vi "subvi(name).vi"(8 "error in":errorcluster) -> (0 "error out":errorcluster, 2 "Button 2":bool, 3 "Cluster ind":T1)   [LabVIEW 2025]
uses:
  Cluster(ctrl2).ctl
  c1a9ddd9-b479-4c69-873f-00e1aee4619d.vi
panel:
  in  "Cluster ind 2":T1
  in  "Button":bool
  in  "Cluster ctrl":T1
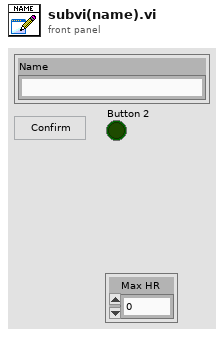
[diagram p1: front panel]
types:
  T1 = typedef "Cluster(ctrl2).ctl" = cluster{"Max HR":i8, "Name":string, "Avg HR":i8}
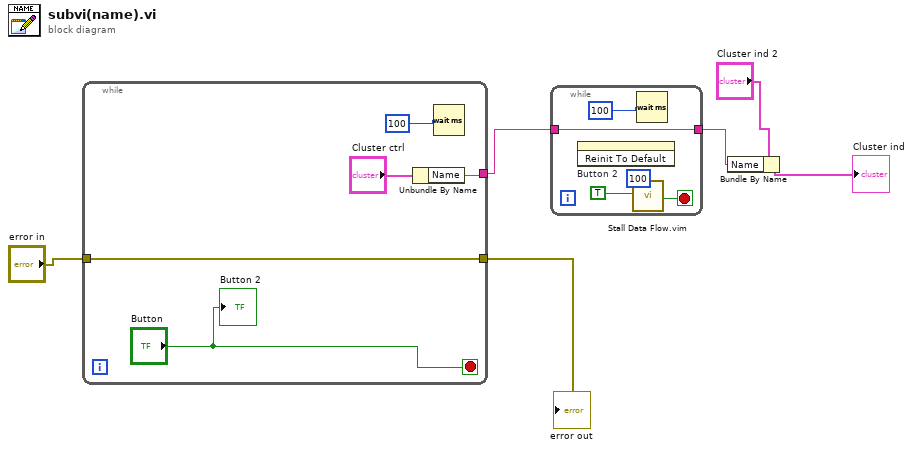
[diagram p0: block diagram]
diagram:
  n1 = while {
    tunnel: [w8] -> w1
    tunnel: [w10] -> w6
    tunnel: "error in" -> [w10]
    stop <- "Button" stop-if-true
    n2 = Unbundle By Name("Cluster ctrl") -> ("Name"=w8:string)
    n3 = Wait (ms)(milliseconds to wait=u32 100) -> ()  [unwired: 1 out]
    "Button 2" <- "Button"
  }
  "error out" <- w6
  n4 = while {
    tunnel: [w16] -> w2
    tunnel: w1 -> [w16]
    stop <- w13 stop-if-true
    n5 = invoke on="Button 2" class="Bool (strict)" method="Reinit To Default"() -> ()  [unwired: 3 in, 3 out]
    n6 = call "Stall Data Flow.vim"("value in"=TRUE, "milliseconds to wait"=u32 100) -> ("value out"=w13:bool)  [unwired: 1 out]
    n7 = Wait (ms)(milliseconds to wait=u32 100) -> ()  [unwired: 1 out]
  }
  n8 = Bundle By Name(cluster="Cluster ind 2", "Name"=w2) -> (→"Cluster ind":T1)
